vi "Read publishedCount.vi"(8 "error in (no error)":errorcluster, 11 "ZM-CM-communication_manager in":refnum<class "ZM-CM-communication_manager.lvclass">) -> (0 "error out":errorcluster, 2 "publishedCount":u32, 3 "ZM-CM-communication_manager out":refnum<class "ZM-CM-communication_manager.lvclass">)   [LabVIEW 2020, in "ZM-CM-communication_manager.lvlib" / "ZM-CM-communication_manager.lvclass"]
doc: "Reads one field of this class's private data. Generated by lvai_create_accessors from the class private data control."
uses:
  ZM-CM-communication_manager.lvclass
  ZM-CM-communication_manager.lvclass/ZM-CM-communication_manager.ctl
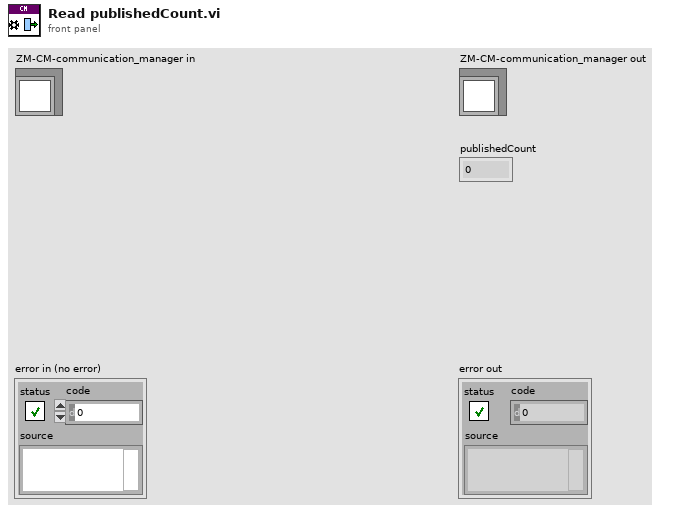
[diagram p1: front panel]
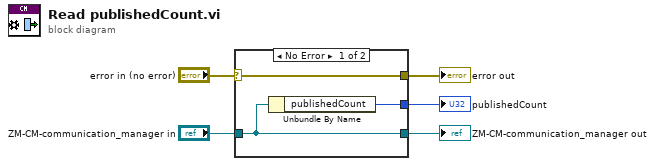
[diagram p0: block diagram]
diagram:
  n1 = case shown="No Error" "error in (no error)" {
    selector: "error in (no error)" -> [w8 w9]
    tunnel: [w8 w9] -> w4
    tunnel: [w7 w10] -> w2
    tunnel: "ZM-CM-communication_manager in" -> [w7 w10]
    tunnel: [w6 _] -> w1
    frame No Error {
      n2 = Unbundle By Name(w7) -> ("publishedCount"=w6:u32)
    }
    frame Error {
    }
  }
  "error out" <- w4
  "ZM-CM-communication_manager out" <- w2
  "publishedCount" <- w1
